vi "CIVI Read Mode.vi"(11 "VISA Resource Name":refnum<visa-resource-name>="TCPIP0::127.0.0.1::5025::SOCKET") -> (0 "error out":errorcluster, 3 "Mode":string)   [LabVIEW 2026]
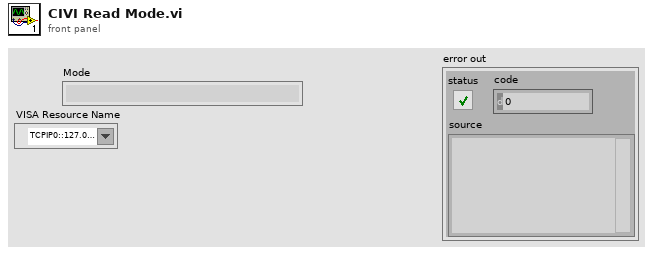
[diagram p1: front panel]
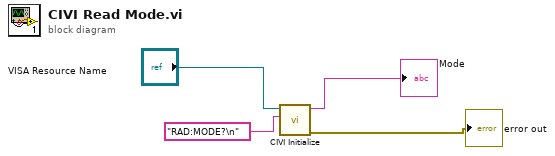
[diagram p0: block diagram]
diagram:
  n1 = call "CIVI Initialize.vi"("write buffer"="RAD:MODE?\n", "VISA Refnum in"="VISA Resource Name") -> ("error out"=→"error out":errorcluster, "read buffer"=→"Mode":string)  [unwired: 8 in]
